vi "Test Black Board.vi"() -> ()   [LabVIEW 2021]
uses:
  Source/Blackboard/Blackboard.lvclass
  Source/Blackboard/Blackboard.lvclass/Blackboard.ctl
  Source/Blackboard/Get Value Type/Get Boolean.vi
  <vilib>/TSA/Abstract Data Classes/Abs_Types/Boolean/Static Write.vi
  <vilib>/TSA/Abstract Data Classes/Abs_Types/Boolean/Static Read.vi
  Source/Blackboard/Support/Index Group.vi
  Source/Blackboard/Support/Index Tags.vi
  <vilib>/TSA/Omni-Bus/Local Bus/Support/Bool/Local Bus_Boolean.lvclass
  C:/Program Files (x86)/National Instruments/LabVIEW 2021/vi.lib/TSA/Abstract Data Classes/Abs_Types/Value/Abs_Value.lvclass
  <vilib>/TSA/Omni-Bus/Local Bus/Support/Initialise DVR's.vi
  <vilib>/TSA/Abstract Data Classes/Abs_Types/Boolean/Abs_Boolean.lvclass
  <vilib>/TSA/Abstract Data Classes/Abs_Types/Value/Abs_Value.lvclass
  <vilib>/TSA/Abstract Data Classes/Abs_Types/Type/Abs_Type.lvclass
  <vilib>/TSA/Omni-Bus/Local Bus/Support/DBL/Local Bus_DBL.lvclass
  <vilib>/TSA/Omni-Bus/Local Bus/Support/SGL/Local Bus_SGL.lvclass
  <vilib>/TSA/Omni-Bus/Local Bus/Support/EXT/Local Bus_EXT.lvclass
  <vilib>/TSA/Omni-Bus/Local Bus/Support/STR/Local Bus_String.lvclass
  <vilib>/TSA/Omni-Bus/Local Bus/Support/Variant/Local Bus_Variant.lvclass
  <vilib>/TSA/Omni-Bus/Local Bus/Support/WFM/Local Bus_Waveform.lvclass
  <vilib>/TSA/Omni-Bus/Local Bus/Support/Time/Local Bus_Time.lvclass
  <vilib>/TSA/Omni-Bus/Local Bus/Support/U8/Local Bus_U8.lvclass
  <vilib>/TSA/Omni-Bus/Local Bus/Support/U16/Local Bus_U16.lvclass
  <vilib>/TSA/Omni-Bus/Local Bus/Support/U32/Local Bus_U32.lvclass
  <vilib>/TSA/Omni-Bus/Local Bus/Support/U64/Local Bus_U64.lvclass
  <vilib>/TSA/Omni-Bus/Local Bus/Support/I8/Local Bus_I8.lvclass
  <vilib>/TSA/Omni-Bus/Local Bus/Support/I16/Local Bus_I16.lvclass
  <vilib>/TSA/Omni-Bus/Local Bus/Support/I32/Local Bus_I32.lvclass
  <vilib>/TSA/Omni-Bus/Local Bus/Support/I64/Local Bus_I64.lvclass
  <vilib>/TSA/Omni-Bus/Local Bus/Support/CSGL/Local Bus_CSGL.lvclass
  <vilib>/TSA/Omni-Bus/Local Bus/Support/CDBL/Local Bus_CDBL.lvclass
  <vilib>/TSA/Omni-Bus/Local Bus/Support/CEXT/Local Bus_CEXT.lvclass
panel:
  in  "Boolean 6":bool
  out "Boolean 5":bool
  in  "Boolean 4":bool
  out "Boolean 3":bool
  in  "stop":bool
  out "Boolean 2":bool
  in  "Boolean":bool
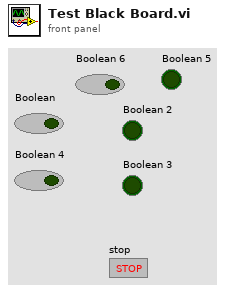
[diagram p1: front panel]
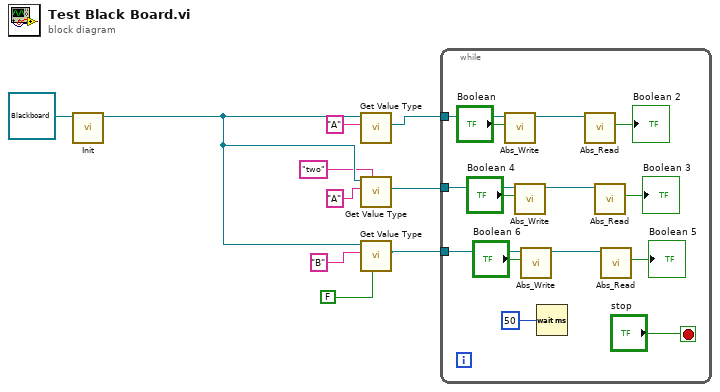
[diagram p0: block diagram]
diagram:
  n1 = call-dynamic "Init.vi"("bt_Blackboard in"=refnum<class "Blackboard.lvclass"> refnum) -> ("bt_Blackboard out"=w6:refnum<class "Blackboard.lvclass">)  [unwired: 9 in, 1 out]
  n2 = call-poly "Get Value Type.vi"("Tag"="A", "Blackboard in"=w6) -> ("Value"=w9:refnum<class "Abs_Boolean.lvclass">)  [unwired: 6 in, 3 out]
  n3 = call-poly "Get Value Type.vi"("Group"="two", "Tag"="A", "Blackboard in"=w6) -> ("Value"=w8:refnum<class "Abs_Boolean.lvclass">)  [unwired: 5 in, 3 out]
  n4 = call-poly "Get Value Type.vi"("Don't Create"=FALSE, "Tag"="B", "Blackboard in"=w6) -> ("Value"=w7:refnum<class "Abs_Boolean.lvclass">)  [unwired: 5 in, 3 out]
  n5 = while {
    tunnel: w9 -> [w24]
    tunnel: w8 -> [w16]
    tunnel: w7 -> [w12]
    stop <- "stop" stop-if-true
    n6 = call-poly <vilib>:"Abs_Write.vi"("Boolean"="Boolean", "Abs_Boolean in"=w24) -> ("Abs_Boolean out"=w22:refnum<class "Abs_Boolean.lvclass">)  [unwired: 8 in, 1 out]
    n7 = call-poly <vilib>:"Abs_Write.vi"("Boolean"="Boolean 4", "Abs_Boolean in"=w16) -> ("Abs_Boolean out"=w18:refnum<class "Abs_Boolean.lvclass">)  [unwired: 8 in, 1 out]
    n8 = call-poly <vilib>:"Abs_Write.vi"("Boolean"="Boolean 6", "Abs_Boolean in"=w12) -> ("Abs_Boolean out"=w14:refnum<class "Abs_Boolean.lvclass">)  [unwired: 8 in, 1 out]
    n9 = Wait (ms)(milliseconds to wait=u32 50) -> ()  [unwired: 1 out]
    n10 = call-poly <vilib>:"Abs_Read.vi"("Abs_Boolean in"=w22) -> ("Boolean"=→"Boolean 2":bool)  [unwired: 8 in, 2 out]
    n11 = call-poly <vilib>:"Abs_Read.vi"("Abs_Boolean in"=w18) -> ("Boolean"=→"Boolean 3":bool)  [unwired: 8 in, 2 out]
    n12 = call-poly <vilib>:"Abs_Read.vi"("Abs_Boolean in"=w14) -> ("Boolean"=→"Boolean 5":bool)  [unwired: 8 in, 2 out]
  }
